vi "AI_Data_Tdms.vi"(11 "error in":errorcluster) -> (15 "error out":errorcluster)   [LabVIEW 2026]
doc: "NI 9203 (8ch, 4-20 mA) current acquisition with DAQmx, per-channel scaling and TDMS save.\nStart: creates the AI current task (0-20 mA range), sample clock timing (finite or continuous) and starts it.\nTimeout (while running): reads N samples/ch as 2D DBL [ch][sample] in A, scales each channel EU = min + (I[mA]-4)/16*(max-min) using row ch of Scale (Min/Max) [min,max], charts it and appends it to the buffer. Finite mode stops the task after one read.\nStop: stops and clears the task.\nSave Data: opens a file dialog (name and folder) and writes the buffered scaled data of every channel to TDMS (group AI Data, channels CH0..CHn).\nClosing the panel ends the VI. Runs only when error in carries no error."
uses:
  <vilib>/DAQmx/miscellaneous.llb/DAQmx Fill In Error Info.vi
panel:
  out "Scaled Data Chart":waveform(dbl)[](graph)
  in  "Scale (Min/Max)":dbl[][](array[numeric])=[[0.0, 100.0], [0.0, 100.0], [0.0, 100.0], [0.0, 100.0], [0.0, 100.0], [0.0, 100.0], [0.0, 100.0], [0.0, 100.0]]
  in  "Save Data":bool
  in  "Stop":bool
  in  "Samples per Channel":i32=100
  in  "Sample Rate (Hz)":dbl=100.0
  in  "Sample Mode":i32(ring)=10123 items=["Finite Samples"=10178, "Continuous Samples"=10123]
  in  "Physical Channels":tag="cDAQ1Mod1/ai0:7"
  in  "Start":bool
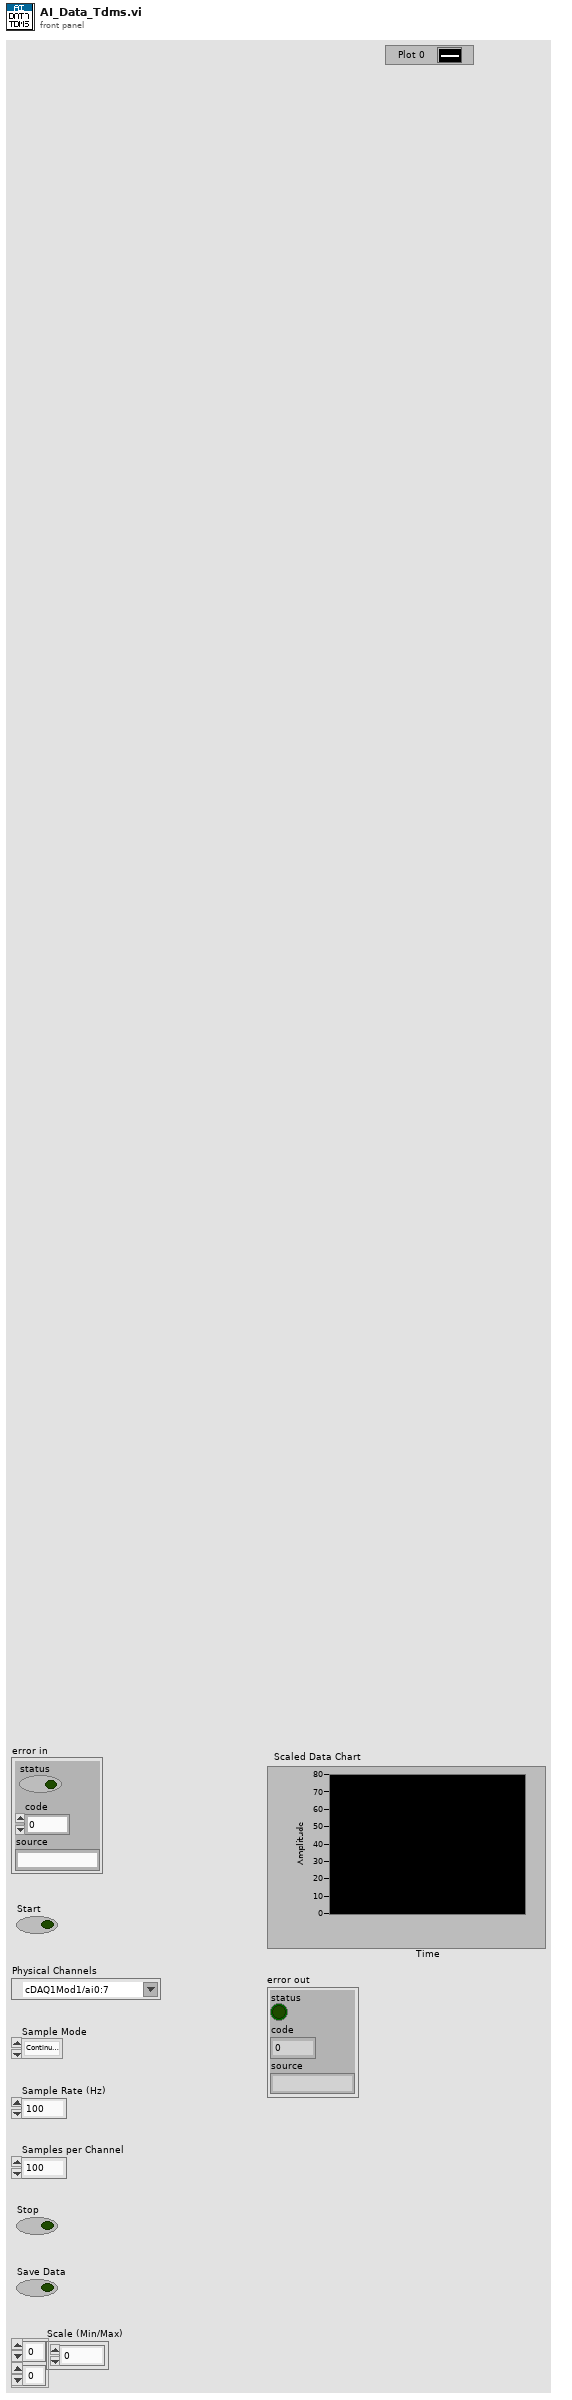
[diagram p1: front panel]
types:
  T1 = enum16{"open", "open or create", "create or replace", "create", "open (read-only)"}
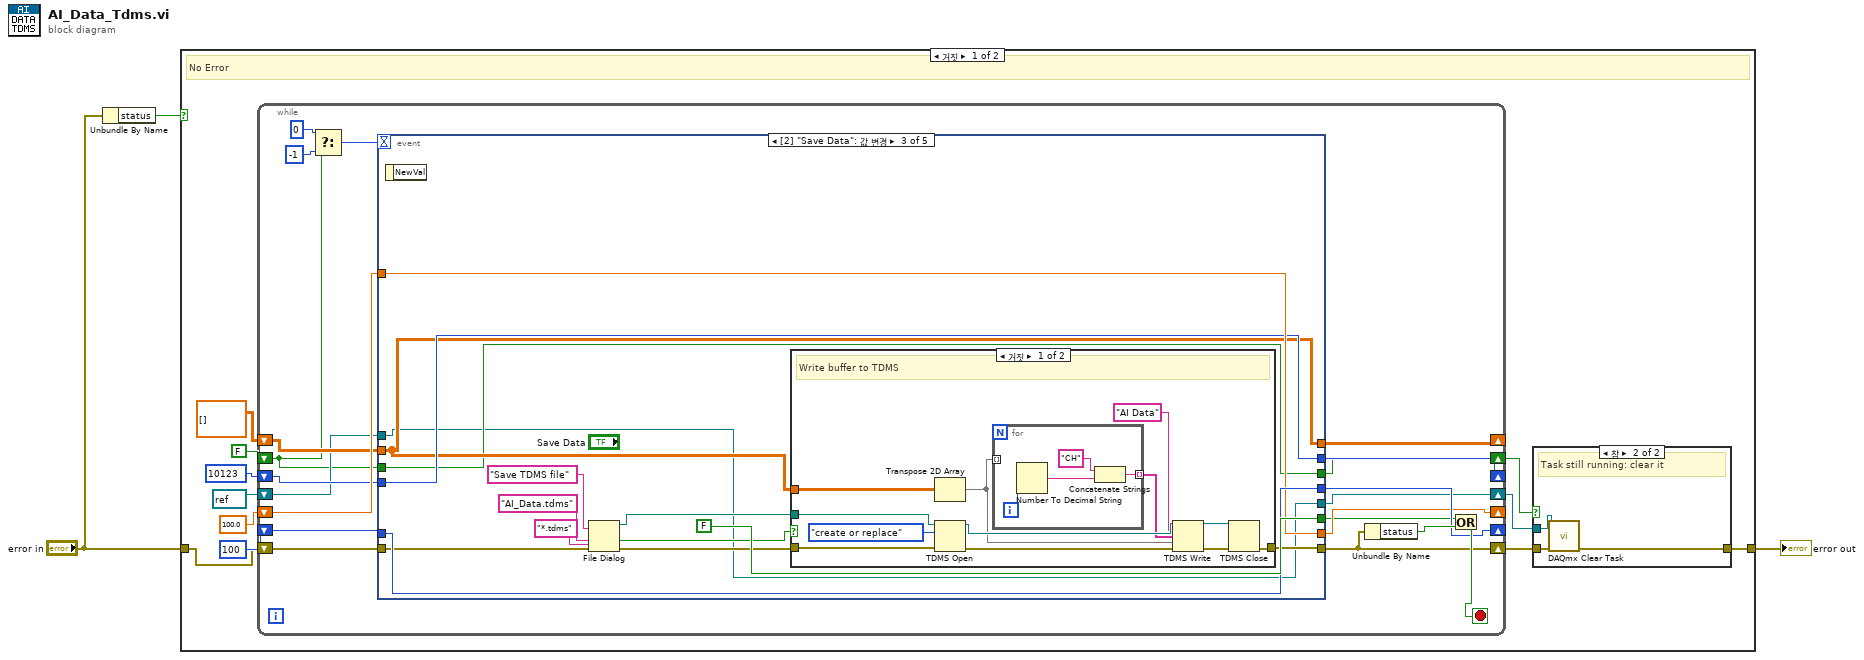
[diagram p0: block diagram]
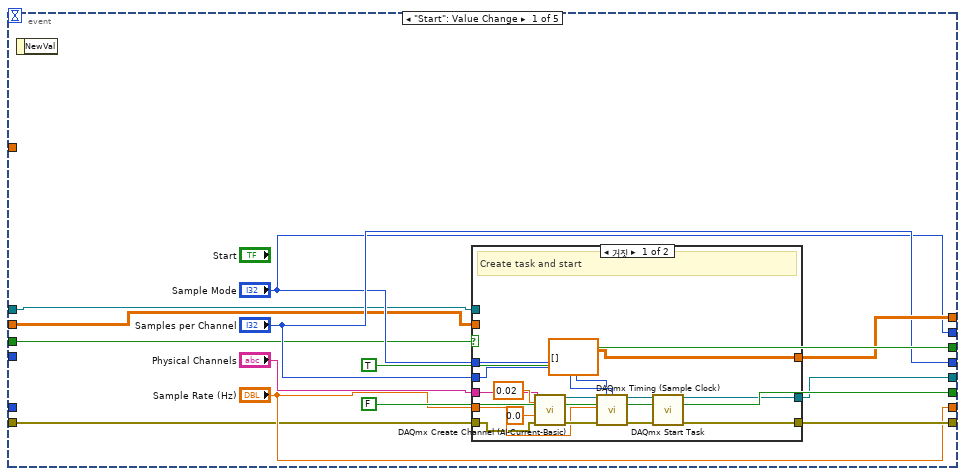
[diagram p3: hidden frame]
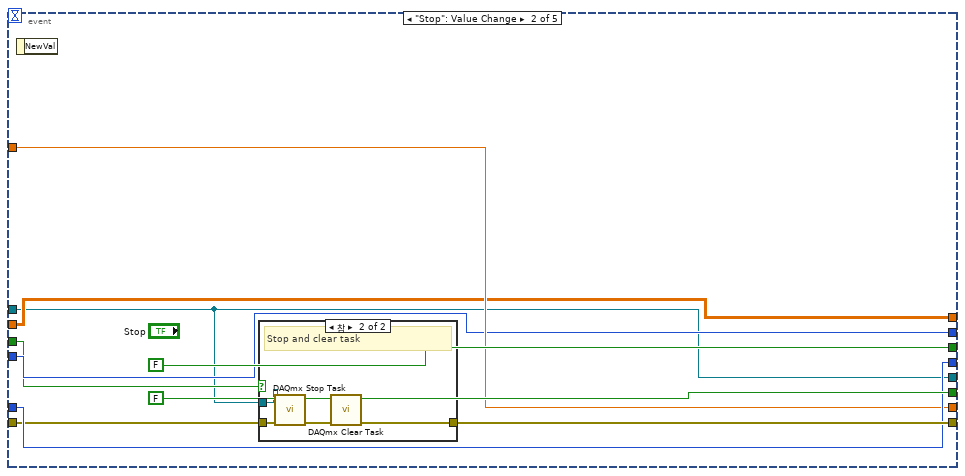
[diagram p5: hidden frame]
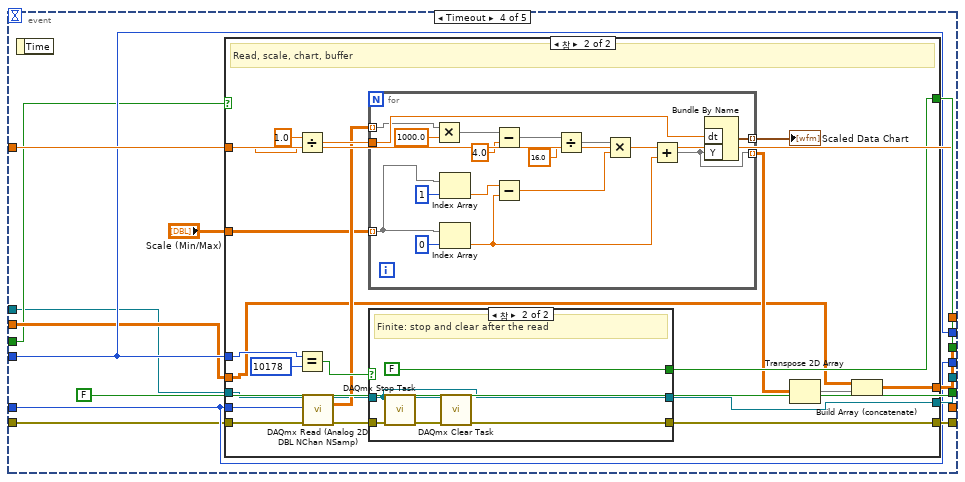
[diagram p8: hidden frame]
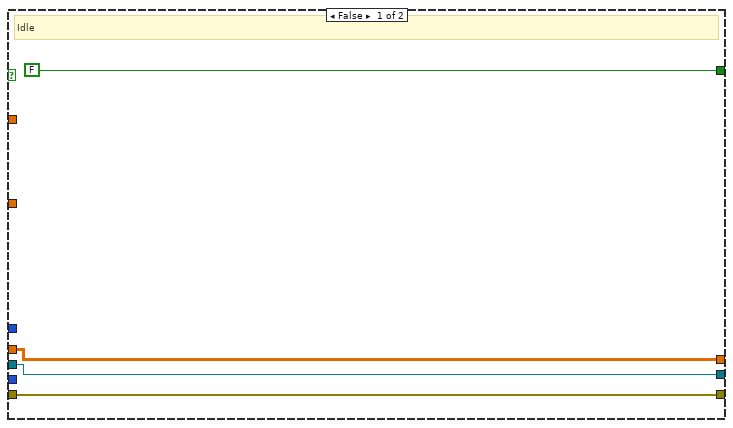
[diagram p9: hidden frame]
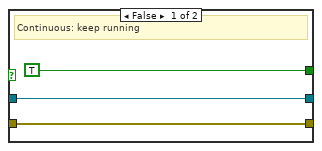
[diagram p10: hidden frame]
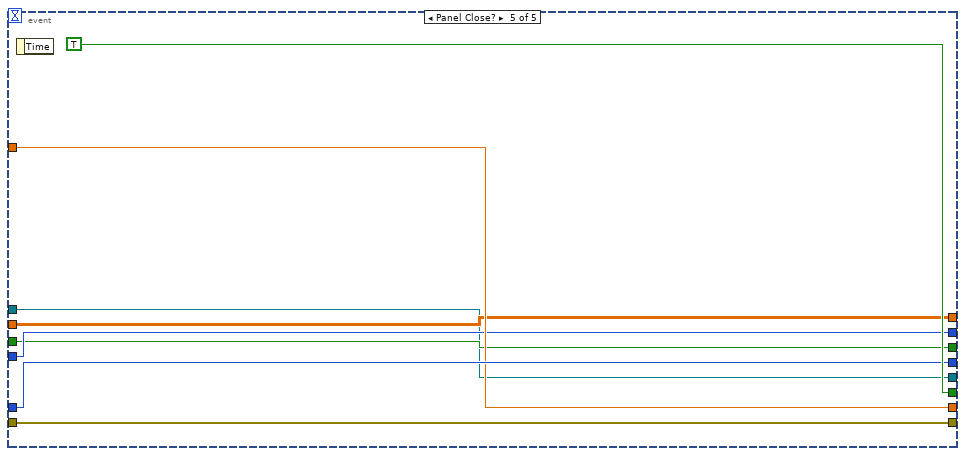
[diagram p11: hidden frame]
diagram:
  n1 = Unbundle By Name("error in") -> ("status"=w2:bool)
  n2 = case shown="거짓" w2 {
    tunnel: "error in" -> [w4 w189]
    tunnel: [w14 w189] -> w3
    frame False {
      # "No Error"
      n3 = while {
        shift-right: [w29] -> w11
        shift-left: refnum<k21> refnum -> [w23]
        shift-right: [w30] -> w12
        shift-left: FALSE -> [w22]
        shift-right: [w31] -> _
        shift-left: dbl[][] [] -> [w24]
        shift-right: [w34] -> _
        shift-left: 10123 -> [w26]
        shift-right: [w35] -> _
        shift-left: 100.0 -> [w27]
        shift-right: [w36] -> _
        shift-left: 100 -> [w28]
        shift-right: [w32] -> w13
        shift-left: w4 -> [w25]
        stop <- w38 stop-if-true
        n4 = Select(t=0, s=w22, f=-1) -> (s? t:f=w21:i32)
        n5 = event shown="[2] \"Save Data\": 값 변경" {
          selector: _ -> [_ _ _ _ _]
          dyn-events: _ -> [_ _ _ _ _]
          timeout: w21 -> [_ _ _ _ _]
          tunnel: [TRUE FALSE w86 w128 w182] -> w30
          tunnel: [FALSE FALSE FALSE FALSE TRUE] -> w33
          tunnel: ["Sample Mode" w73 w89 w121 w185] -> w34
          tunnel: ["Sample Rate (Hz)" w74 w90 w122 w186] -> w35
          tunnel: ["Samples per Channel" w75 w91 w123 w187] -> w36
          tunnel: w23 -> [w39 w69 w85 w117 w181]
          tunnel: w22 -> [w40 w70 w86 w118 w182]
          tunnel: w24 -> [w41 w71 w87 w119 w183]
          tunnel: w26 -> [_ w73 w89 w121 w185]
          tunnel: w27 -> [_ w74 w90 w122 w186]
          tunnel: w28 -> [_ w75 w91 w123 w187]
          tunnel: w25 -> [w42 w72 w88 w120 w184]
          tunnel: [w47 w69 w85 w125 w181] -> w29
          tunnel: [w49 w71 w87 w127 w183] -> w31
          tunnel: [w48 w76 w98 w126 w184] -> w32
          event "Start": Value Change {
            n6 = event-data() -> ()  [unwired: 1 in, 1 out]
            n7 = case shown="거짓" w40 {
              tunnel: "Physical Channels" -> [w53 _]
              tunnel: "Sample Mode" -> [w54 _]
              tunnel: "Sample Rate (Hz)" -> [w55 _]
              tunnel: "Samples per Channel" -> [w56 _]
              tunnel: w39 -> [_ w66]
              tunnel: w41 -> [_ w68]
              tunnel: w42 -> [w52 w67]
              tunnel: [w63 w66] -> w47
              tunnel: [dbl[][] [] w68] -> w49
              tunnel: [w64 w67] -> w48
              frame False {
                # "Create task and start"
                n8 = call <vilib>:"DAQmx Create Channel (AI-Current-Basic).vi"("maximum value"=0.02, "minimum value"=0.0, "physical channels"=w53, "error in"=w52) -> ("task out"=w59:refnum<k21>, "error out"=w60:errorcluster)  [unwired: 10 in]
                n9 = call <vilib>:"DAQmx Timing (Sample Clock).vi"("task/channels in"=w59, "sample mode"=w54, "samples per channel"=w56, "rate"=w55, "error in"=w60) -> ("task out"=w61:refnum<k21>, "error out"=w62:errorcluster)  [unwired: 9 in]
                n10 = call <vilib>:"DAQmx Start Task.vi"("task/channels in"=w61, "error in"=w62) -> ("task out"=w63:refnum<k21>, "error out"=w64:errorcluster)  [unwired: 12 in]
              }
              frame True {
                # "Already running"
              }
            }
          }
          event "Stop": Value Change {
            n11 = event-data() -> ()  [unwired: 1 in, 1 out]
            n12 = case shown="참" w70 {
              tunnel: w69 -> [_ w80]
              tunnel: w72 -> [w79 w81]
              tunnel: [w79 w84] -> w76
              frame False {
                # "Not running"
              }
              frame True {
                # "Stop and clear task"
                n13 = call <vilib>:"DAQmx Stop Task.vi"("task/channels in"=w80, "error in"=w81) -> ("task out"=w82:refnum<k21>, "error out"=w83:errorcluster)  [unwired: 12 in]
                n14 = call <vilib>:"DAQmx Clear Task.vi"("task in"=w82, "error in"=w83) -> ("error out"=w84:errorcluster)  [unwired: 13 in]
              }
            }
          }
          event "Save Data": Value Change {
            n15 = event-data() -> ()  [unwired: 1 in, 1 out]
            n16 = File Dialog(6:"*.tdms", 7:"Save TDMS file", 8:w88, 9:"AI_Data.tdms") -> (0:w97:errorcluster, 1:w96:bool, 3:w95:path)  [unwired: 3 in, 1 out]
            n17 = case shown="거짓" w96 {
              tunnel: w87 -> [w102 _]
              tunnel: w95 -> [w100 _]
              tunnel: w97 -> [w101 w116]
              tunnel: [w111 w116] -> w98
              frame False {
                # "Write buffer to TDMS"
                n18 = Transpose 2D Array(2D array=w102) -> (transposed array=w103:dbl[][])
                n19 = TDMS Open(8:w101, 10:T1."create or replace" ("operation"), 11:w100) -> (0:w108:errorcluster, 3:w107:refnum<k34>)  [unwired: 4 in]
                n20 = for {
                  tunnel: [w115] -> w104 mode=indexing
                  tunnel: w103 -> [_] mode=indexing
                  i -> [w112]
                  n21 = Number To Decimal String(number=w112) -> (decimal integer string=w114:string)  [unwired: 1 in]
                  n22 = Concatenate Strings("CH", w114) -> (w115:string)
                }
                n23 = TDMS Write(0:w107, 5:"AI Data", 7:w104, 9:w103, 11:w108) -> (4:w109:refnum<k34>, 15:w110:errorcluster)  [unwired: 1 in, 2 out]
                n24 = TDMS Close(8:w110, 11:w109) -> (0:w111:errorcluster)  [unwired: 1 out]
              }
              frame True {
                # "Dialog cancelled"
              }
            }
          }
          event Timeout {
            n25 = event-data() -> ()  [unwired: 1 in, 1 out]
            n26 = case shown="참" w118 {
              tunnel: "Scale (Min/Max)" -> [_ w137]
              tunnel: [FALSE w154] -> w128
              tunnel: w117 -> [w130 w134]
              tunnel: w119 -> [w132 w136]
              tunnel: w123 -> [_ w138]
              tunnel: w122 -> [_ w139]
              tunnel: w121 -> [_ w140]
              tunnel: w120 -> [w131 w135]
              tunnel: [w130 w152] -> w125
              tunnel: [w131 w153] -> w126
              tunnel: [w132 w149] -> w127
              frame False {
                # "Idle"
              }
              frame True {
                # "Read, scale, chart, buffer"
                n27 = Divide(x=1.0, y=w139) -> (x/y=w145:dbl)
                n28 = Equal?(x=w140, y=10178) -> (x = y?=w151:bool)
                n29 = call <vilib>:"DAQmx Read (Analog 2D DBL NChan NSamp).vi"("task/channels in"=w134, "number of samples per channel"=w138, "error in"=w135) -> ("task out"=w141:refnum<k21>, "data"=w142:dbl[][], "error out"=w143:errorcluster)  [unwired: 10 in]
                n30 = for {
                  tunnel: w137 -> [w165] mode=indexing
                  tunnel: w145 -> [w166]
                  tunnel: w142 -> [w164] mode=indexing
                  tunnel: [w179] -> w146 mode=indexing
                  tunnel: [w180] -> w147 mode=indexing
                  n31 = Multiply(x=w164, y=1000.0) -> (x*y=w174:dbl[])
                  n32 = Index Array(array=w165, index=1) -> (element=w170:dbl)
                  n33 = Index Array(array=w165, index=0) -> (element=w169:dbl)
                  n34 = Subtract(x=w174, y=4.0) -> (x-y=w175:dbl[])
                  n35 = Subtract(x=w170, y=w169) -> (x-y=w177:dbl)
                  n36 = Divide(x=w175, y=16.0) -> (x/y=w176:dbl[])
                  n37 = Multiply(x=w176, y=w177) -> (x*y=w178:dbl[])
                  n38 = Add(x=w178, y=w169) -> (x+y=w179:dbl[])
                  n39 = Bundle By Name("dt"=w166, "Y"=w179) -> (w180:waveform(dbl))  [unwired: 1 in]
                }
                "Scaled Data Chart" <- w147
                n40 = case shown="참" w151 {
                  tunnel: [TRUE FALSE] -> w154
                  tunnel: w141 -> [w155 w158]
                  tunnel: w143 -> [w156 w159]
                  tunnel: [w155 w158] -> w152
                  tunnel: [w156 w162] -> w153
                  frame False {
                    # "Continuous: keep running"
                  }
                  frame True {
                    # "Finite: stop and clear after the read"
                    n41 = call <vilib>:"DAQmx Stop Task.vi"("task/channels in"=w158, "error in"=w159) -> ("task out"=w160:refnum<k21>, "error out"=w161:errorcluster)  [unwired: 12 in]
                    n42 = call <vilib>:"DAQmx Clear Task.vi"("task in"=w160, "error in"=w161) -> ("error out"=w162:errorcluster)  [unwired: 13 in]
                  }
                }
                n43 = Transpose 2D Array(2D array=w146) -> (transposed array=w148:dbl[][])
                n44 = Build Array (concatenate)(w136, w148) -> (w149:dbl[][])
              }
            }
          }
          event Panel Close? {
            n45 = event-data() -> ()  [unwired: 2 in, 1 out]
            n46 = event-data() -> ()  [unwired: 1 in, 1 out]
          }
        }
        n47 = Unbundle By Name(w32) -> ("status"=w37:bool)
        n48 = Or(x=w33, y=w37) -> (x .or. y?=w38:bool)
      }
      n49 = case shown="참" w12 {
        tunnel: w11 -> [_ w16]
        tunnel: w13 -> [w15 w17]
        tunnel: [w15 w18] -> w14
        frame False {
        }
        frame True {
          # "Task still running: clear it"
          n50 = call <vilib>:"DAQmx Clear Task.vi"("task in"=w16, "error in"=w17) -> ("error out"=w18:errorcluster)  [unwired: 13 in]
        }
      }
    }
    frame True {
      # "Error"
    }
  }
  "error out" <- w3
